vi "SeqEditor_initloading.vi"(8 "error in (no error)":errorcluster, 11 "NLTest in":refnum<class "NLTest.lvclass">) -> (0 "error out":errorcluster, 3 "NLTest out":refnum<class "NLTest.lvclass">)   [LabVIEW 2017, in "NLTest.lvclass"]
uses:
  NLTest.lvclass
  VISTEP_class_steptestclass.ctl
  VISTEP.ctl
  VISTEP_class_INOUTPUT.ctl
  VISTEP_class_INOUTPUT_TYPE.ctl
  VISTEP_class_NumberTest_OP.ctl
  NLTest.lvclass/NLTest.ctl
panel:
  in  "NumberTest_OP":T1
  out "debug":T2[](array[typedef])
  in  "步骤类型":T5
  # "Y Y  LL"
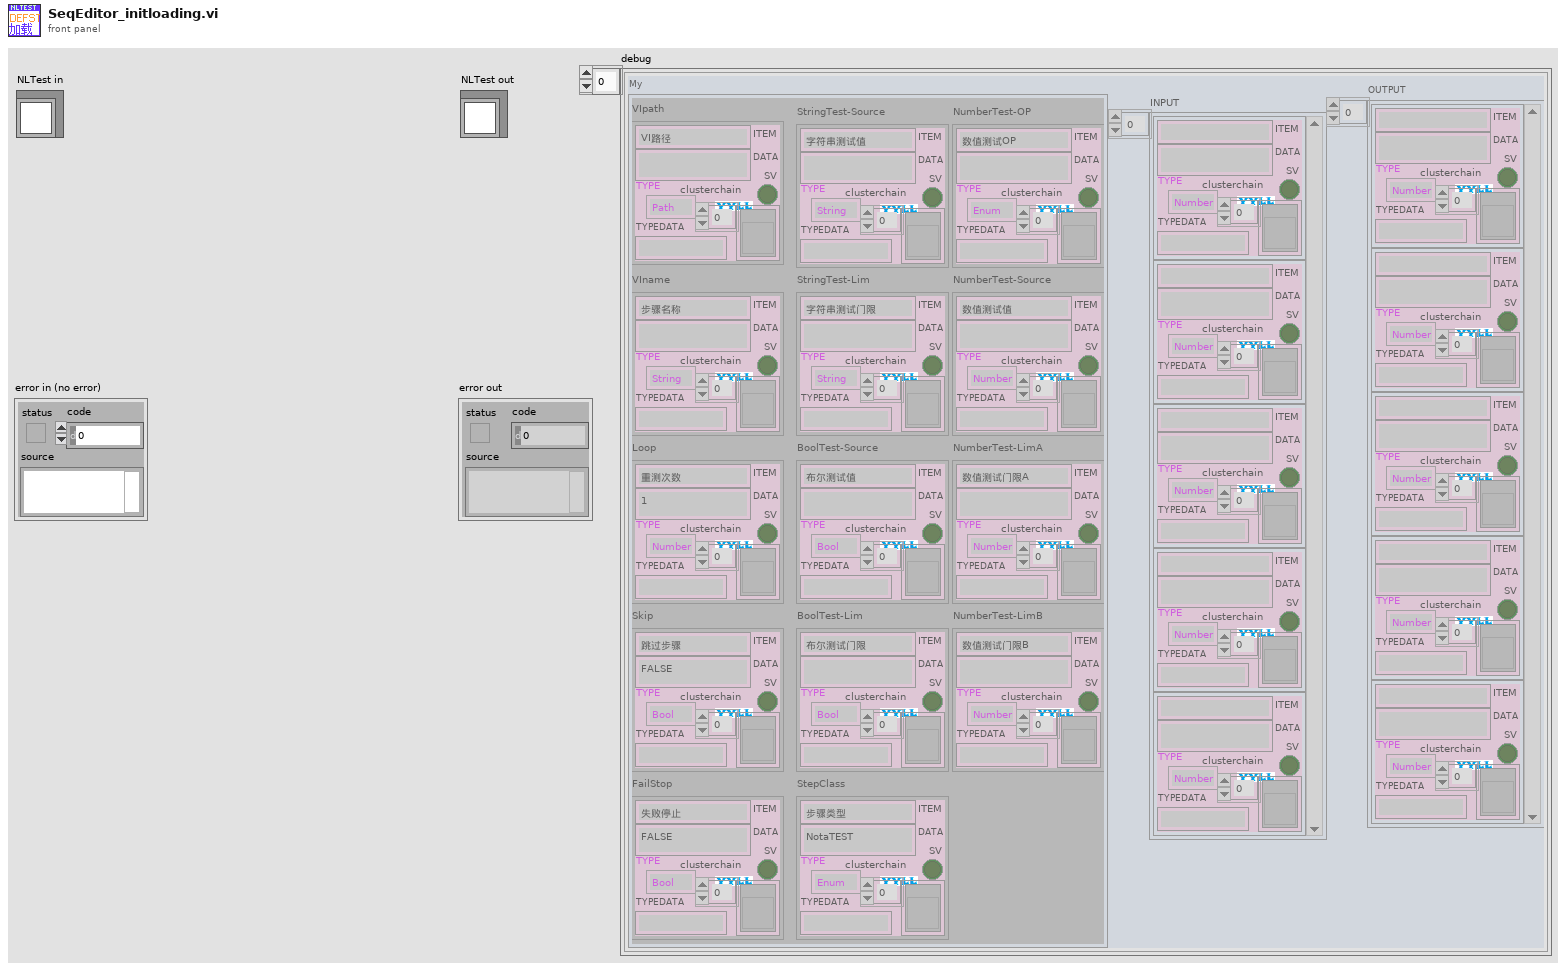
[diagram p1: front panel]
types:
  T1 = typedef "NLTest.lvclass/VISTEP_class_NumberTest_OP.ctl" = enum16{"X=A", "X!=A", "X<=A", "X>=A", "A<=X<=B", "X<=A && B<=X", "X<=A || B<=X"}
  T2 = typedef "NLTest.lvclass/VISTEP.ctl" = cluster{"My":cluster{"VIpath":T3, "VIname":T3, "Loop":T3, "Skip":T3, "FailStop":T3, "StepClass":T3, "StringTest-Source":T3, "StringTest-Lim":T3, "BoolTest-Source":T3, "BoolTest-Lim":T3, "NumberTest-OP":T3, "NumberTest-Source":T3, "NumberTest-LimA":T3, "NumberTest-LimB":T3}, "INPUT":T3[], "OUTPUT":T3[]}
  T3 = typedef "NLTest.lvclass/VISTEP_class_INOUTPUT.ctl" = cluster{"ITEM":string, "DATA":string, "TYPE":T4, "TYPEDATA":string, "SV":bool, "clusterchain":refnum<vi>[]}
  T4 = typedef "NLTest.lvclass/VISTEP_class_INOUTPUT_TYPE.ctl" = enum16{"Number", "String", "Bool", "Enum", "Path", "VISA", "NA"}
  T5 = typedef "NLTest.lvclass/VISTEP_class_steptestclass.ctl" = enum16{"NotaTest", "StringTest", "BoolTest", "NumberTest", "NULL"}
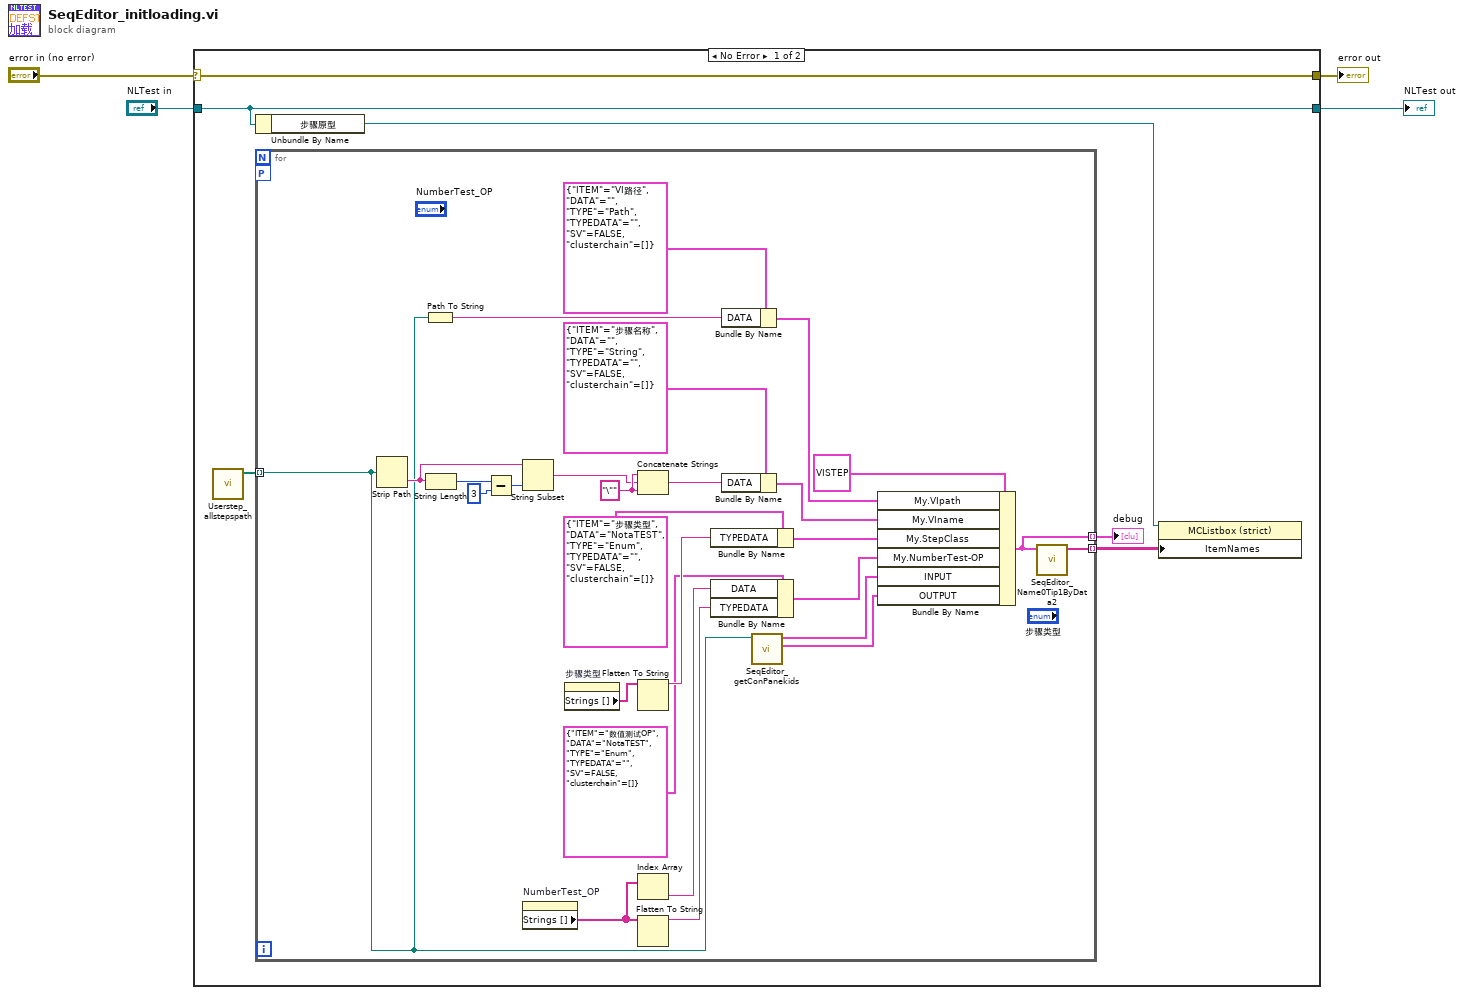
[diagram p0: block diagram]
diagram:
  n1 = case shown="No Error" "error in (no error)" {
    selector: "error in (no error)" -> [w10 w39]
    tunnel: [w10 w39] -> w3
    tunnel: [w7 w38] -> w1
    tunnel: "NLTest in" -> [w7 w38]
    frame No Error {
      n2 = call "Userstep_allstepspath.vi"() -> ("Array"=w9:path[])  [unwired: 11 in]
      n3 = Unbundle By Name(w7) -> ("步骤原型"=w6:refnum<vi>)
      n4 = for {
        tunnel: w9 -> [w31] mode=indexing
        tunnel: [w11] -> w8 mode=indexing
        workers-P: _ -> [_]
        tunnel: [w12] -> w5 mode=indexing
        w14 = "\"" ("string")
        n5 = Strip Path(path=w31) -> (name=w33:string)  [unwired: 1 out]
        n6 = Path To String(path=w31) -> (string=w30:string)
        n7 = String Length(string=w33) -> (length=w37:i32)
        n8 = Subtract(x=w37, y=3) -> (x-y=w35:i32)
        n9 = String Subset(string=w33, length (rest)=w35) -> (substring=w13:string)  [unwired: 1 in]
        n10 = property on="NumberTest_OP" class="Enum (strict)"() -> ("Strings []"=w17:string[])  [unwired: 2 in, 2 out]
        n11 = property on="步骤类型" class="Enum (strict)"() -> ("Strings []"=w21:string[])  [unwired: 2 in, 2 out]
        n12 = Concatenate Strings(w14, w13, w14) -> (w15:string)
        n13 = Flatten To String(anything=w21) -> (data string=w20:string)  [unwired: 3 in, 2 out]
        n14 = Index Array(array=w17) -> (element=w16:string)  [unwired: 1 in]
        n15 = Flatten To String(anything=w17) -> (data string=w19:string)  [unwired: 3 in, 2 out]
        n16 = Bundle By Name(cluster=T3 {"ITEM"="步骤类型", "DATA"="NotaTEST", "TYPE"=enum."Enum", "TYPEDATA"="", "SV"=FALSE, "clusterchain"=[]} ("Cluster"), "TYPEDATA"=w20) -> (w27:T3)
        n17 = Bundle By Name(cluster=T3 {"ITEM"="数值测试OP", "DATA"="NotaTEST", "TYPE"=enum."Enum", "TYPEDATA"="", "SV"=FALSE, "clusterchain"=[]} ("Cluster"), "DATA"=w16, "TYPEDATA"=w19) -> (w26:T3)
        n18 = Bundle By Name(cluster=T3 {"ITEM"="VI路径", "DATA"="", "TYPE"=enum."Path", "TYPEDATA"="", "SV"=FALSE, "clusterchain"=[]} ("Cluster"), "DATA"=w30) -> (w29:T3)
        n19 = Bundle By Name(cluster=T3 {"ITEM"="步骤名称", "DATA"="", "TYPE"=enum."String", "TYPEDATA"="", "SV"=FALSE, "clusterchain"=[]} ("Cluster"), "DATA"=w15) -> (w28:T3)
        n20 = call "SeqEditor_getConPanekids.vi"("steppath"=w31) -> ("OUTPUT"=w23:T3[], "INPUT"=w24:T3[])  [unwired: 9 in]
        n21 = Bundle By Name(cluster=T2 {"My"={"VIpath"={"ITEM"="VI路径", "DATA"="\"\"", "TYPE"=enum."Path", "TYPEDATA"="", "SV"=FALSE, "clusterchain"=[]}, "VIname"={"ITEM"="步骤名称", "DATA"="\"\"", "TYPE"=enum."String", "TYPEDATA"="", "SV"=FALSE, "clusterchain"=[]}, "Loop"={"ITEM"="重测次数", "DATA"="1", "TYPE"=enum."Number", "TYPEDATA"="", "SV"=FALSE, "clusterchain"=[]}, "Skip"={"ITEM"="跳过步骤", "DATA"="FALSE", "TYPE"=enum."Bool", "TYPEDATA"="", "SV"=FALSE, "clusterchain"=[]}, "FailStop"={"ITEM"="失败停止", "DATA"="FALSE", "TYPE"=enum."Bool", "TYPEDATA"="", "SV"=FALSE, "clusterchain"=[]}, "StepClass"={"ITEM"="步骤类型", "DATA"="NotaTEST", "TYPE"=enum."Enum", "TYPEDATA"="", "SV"=FALSE, "clusterchain"=[]}, "StringTest-Source"={"ITEM"="字符串测试值", "DATA"="\"\"", "TYPE"=enum."String", "TYPEDATA"="", "SV"=FALSE, "clusterchain"=[]}, "StringTest-Lim"={"ITEM"="字符串测试门限", "DATA"="\"\"", "TYPE"=enum."String", "TYPEDATA"="", "SV"=FALSE, "clusterchain"=[]}, "BoolTest-Source"={"ITEM"="布尔测试值", "DATA"="TRUE", "TYPE"=enum."Bool", "TYPEDATA"="", "SV"=FALSE, "clusterchain"=[]}, "BoolTest-Lim"={"ITEM"="布尔测试门限", "DATA"="TRUE", "TYPE"=enum."Bool", "TYPEDATA"="", "SV"=FALSE, "clusterchain"=[]}, "NumberTest-OP"={"ITEM"="数值测试OP", "DATA"="NotaTEST", "TYPE"=enum."Enum", "TYPEDATA"="", "SV"=FALSE, "clusterchain"=[]}, "NumberTest-Source"={"ITEM"="数值测试值", "DATA"="0", "TYPE"=enum."Number", "TYPEDATA"="", "SV"=FALSE, "clusterchain"=[]}, "NumberTest-LimA"={"ITEM"="数值测试门限A", "DATA"="0", "TYPE"=enum."Number", "TYPEDATA"="", "SV"=FALSE, "clusterchain"=[]}, "NumberTest-LimB"={"ITEM"="数值测试门限B", "DATA"="0", "TYPE"=enum."Number", "TYPEDATA"="", "SV"=FALSE, "clusterchain"=[]}}, "INPUT"=[], "OUTPUT"=[]} ("步骤结构"), "My.VIpath"=w29, "My.VIname"=w28, "My.StepClass"=w27, "My.NumberTest-OP"=w26, "INPUT"=w24, "OUTPUT"=w23) -> (w12:T2)
        n22 = call "SeqEditor_Name0Tip1ByData2.vi"("output cluster"=w12) -> ("Array"=w11:string[])  [unwired: 10 in]
      }
      "debug" <- w5
      n23 = property on="Property Node" class="MCListbox (strict)"(reference=w6, "ItemNames"=w8) -> ()  [unwired: 1 in, 2 out]
    }
    frame Error {
    }
  }
  "error out" <- w3
  "NLTest out" <- w1
